vi "Learn form template.vi"(8 "error in (no error)":errorcluster, 11 "Template Image":T1) -> (0 "error out":errorcluster, 3 "Refnum out":T1)   [LabVIEW 2014]
uses:
  <vilib>/vision/Image Controls.llb/IMAQ Image.ctl
  <vilib>/vision/NI_Vision_Development_Module.lvlib
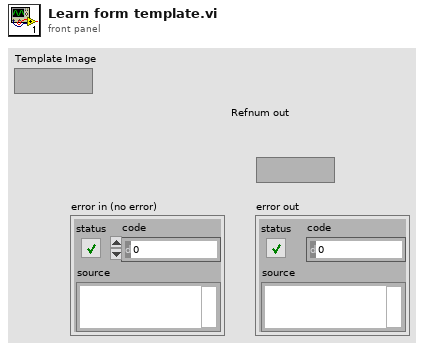
[diagram p1: front panel]
types:
  T1 = typedef "IMAQ Image.ctl" = refnum<image>
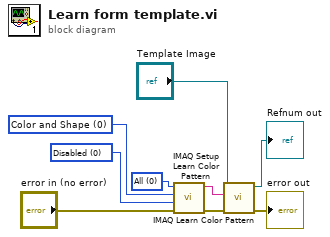
[diagram p0: block diagram]
diagram:
  w5 = u32 0 items=["Disabled", "Ignore Black", "Ignore White", "Ignore Black and White"] ("Ignore Black and White")
  w4 = u32 0 items=["Color and Shape", "Color", "Shape "] ("Feature Mode")
  w3 = u32 0 items=["All", "Shift Information", "Rotation Information"] ("Learn Mode")
  n1 = call "IMAQ Setup Learn Color Pattern"("error in (no error)"="error in (no error)", "Ignore Black and White"=w5, "Feature Mode"=w4, "Learn Mode"=w3) -> ("error out"=w2:errorcluster, "Learn Color Pattern Setup Data"=w6:string)  [unwired: 6 in]
  n2 = call "IMAQ Learn Color Pattern"("error in (no error)"=w2, "Learn Color Pattern Setup Data"=w6, "Image"="Template Image") -> ("error out"=→"error out":errorcluster, "Template Image Out"=→"Refnum out":T1)  [unwired: 7 in]
